vi "init Call Box Device.vi"(8 "error in (no error)":errorcluster, 9 "Device - Protocol":T1, 10 "VISA Address":refnum<visa-resource-name>, 11 "Anritsu Call Box in":refnum<class "Anritsu Call Box.lvclass">) -> (0 "error out":errorcluster, 2 "Connected":bool, 3 "Anritsu Call Box out":refnum<class "Anritsu Call Box.lvclass">)   [LabVIEW 2023, in "ANRITSU Call Box.lvlib" / "Anritsu Call Box.lvclass"]
uses:
  Anritsu Call Box.lvclass
  Type Definition/Call Device - Protocol Type Selector.ctl
  ANRITSU Call Box.lvlib
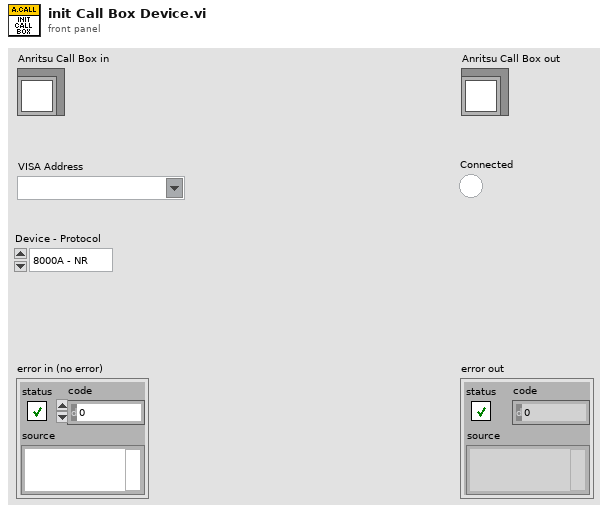
[diagram p1: front panel]
types:
  T1 = typedef "ANRITSU Call Box.lvlib/Call Device - Protocol Type Selector.ctl" = enum16{"8000A - NR", "8000A - LTE", "882xC - LTE"}
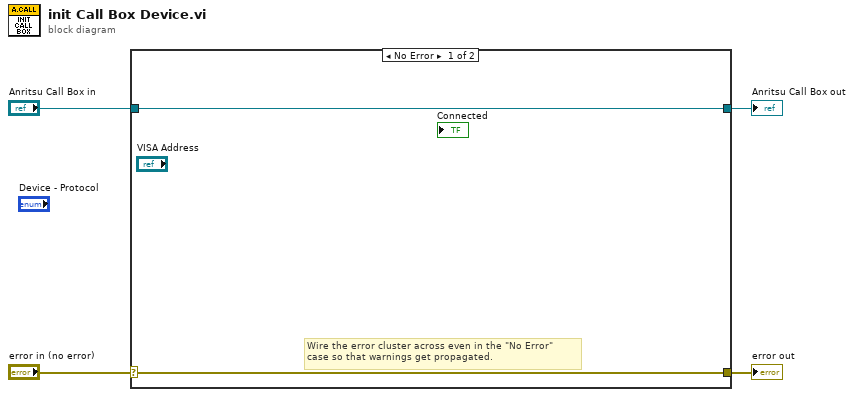
[diagram p0: block diagram]
diagram:
  n1 = case shown="No Error" "error in (no error)" {
    selector: "error in (no error)" -> [w5 w8]
    tunnel: [w5 w8] -> w3
    tunnel: [w6 w7] -> w1
    tunnel: "Anritsu Call Box in" -> [w6 w7]
    frame No Error {
      # "Wire the error cluster across even in the \"No Error\"\ncase so that warnings get propagated."
    }
    frame Error {
    }
  }
  "error out" <- w3
  "Anritsu Call Box out" <- w1
